vi "RemoteVI Answer Control Frame.vi"(0 "connection":u32, 1 "close code":u16=1000, 2 "closed?":bool, 5 "ping?":bool, 7 "payload":string, 9 "close?":bool) -> (4 "closed out":bool)   [LabVIEW 2020, in "RemoteVI.lvlib"]
doc: "Answers a client's control frame (docs\\protocol.md section 4): a ping with a pong carrying payload; close? with a close frame carrying close code, after which the client is closed. Writes with a 2 s timeout; a failed pong write closes the client too. connection is the TCP connection refnum type-cast to U32."
uses:
  RemoteVI.lvlib
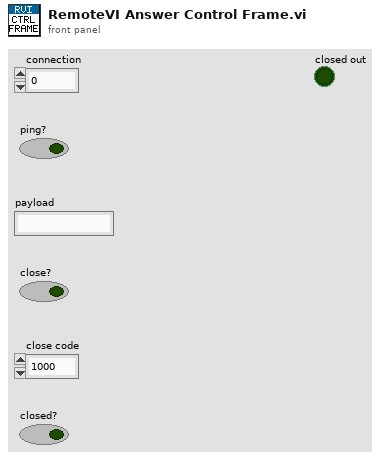
[diagram p1: front panel]
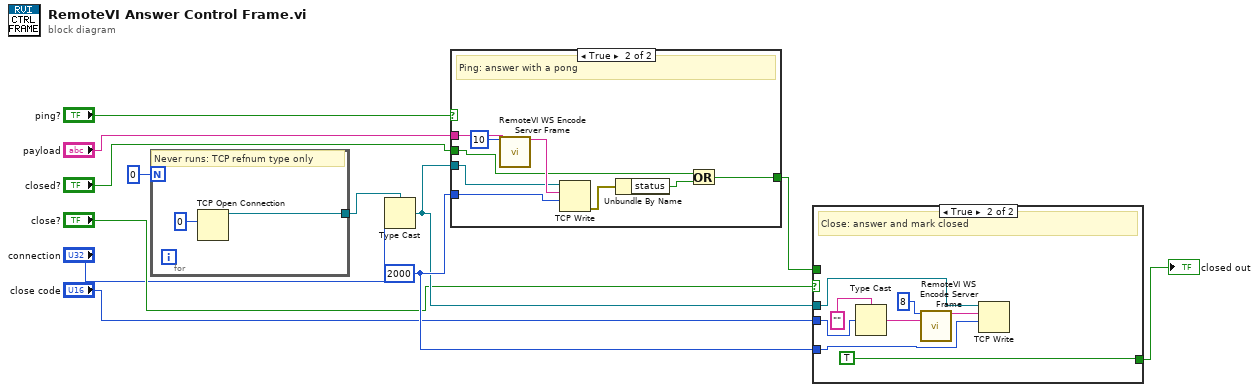
[diagram p0: block diagram]
diagram:
  w10 = 2000
  n1 = for {
    N: 0 -> [_]
    tunnel: [w14] -> w8
    # "Never runs: TCP refnum type only"
    n2 = TCP Open Connection(remote port or service name=u16 0) -> (connection ID=w14:refnum<k5>)  [unwired: 4 in, 1 out]
  }
  n3 = Type Cast(type=w8, x="connection") -> (*(type *) &x=w9:refnum<k5>)
  n4 = case shown="True" "ping?" {
    tunnel: "payload" -> [_ w16]
    tunnel: "closed?" -> [w15 w18]
    tunnel: w10 -> [_ w19]
    tunnel: w9 -> [_ w17]
    tunnel: [w15 w24] -> w11
    frame False {
    }
    frame True {
      # "Ping: answer with a pong"
      n5 = call "RemoteVI WS Encode Server Frame.vi"("opcode"=u8 10, "payload"=w16) -> ("frame"=w21:string)  [unwired: 13 in]
      n6 = TCP Write(connection ID=w17, data in=w21, 9:w19) -> (error out=w22:errorcluster)  [unwired: 1 in, 2 out]
      n7 = Unbundle By Name(w22) -> ("status"=w23:bool)
      n8 = Or(x=w18, y=w23) -> (x .or. y?=w24:bool)
    }
  }
  n9 = case shown="True" "close?" {
    tunnel: "close code" -> [_ w26]
    tunnel: w10 -> [_ w28]
    tunnel: [w25 TRUE] -> w12
    tunnel: w9 -> [_ w27]
    tunnel: w11 -> [w25 _]
    frame False {
    }
    frame True {
      # "Close: answer and mark closed"
      n10 = Type Cast(type="", x=w26) -> (*(type *) &x=w30:string)
      n11 = call "RemoteVI WS Encode Server Frame.vi"("opcode"=u8 8, "payload"=w30) -> ("frame"=w32:string)  [unwired: 13 in]
      n12 = TCP Write(connection ID=w27, data in=w32, 9:w28) -> ()  [unwired: 1 in, 3 out]
    }
  }
  "closed out" <- w12
